vi "hamming encoder.vi"(10 "number of control bits":i32, 11 "message":u8) -> (3 "output array":bool[](array[boolean]))   [LabVIEW 2025]
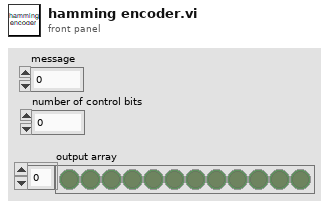
[diagram p1: front panel]
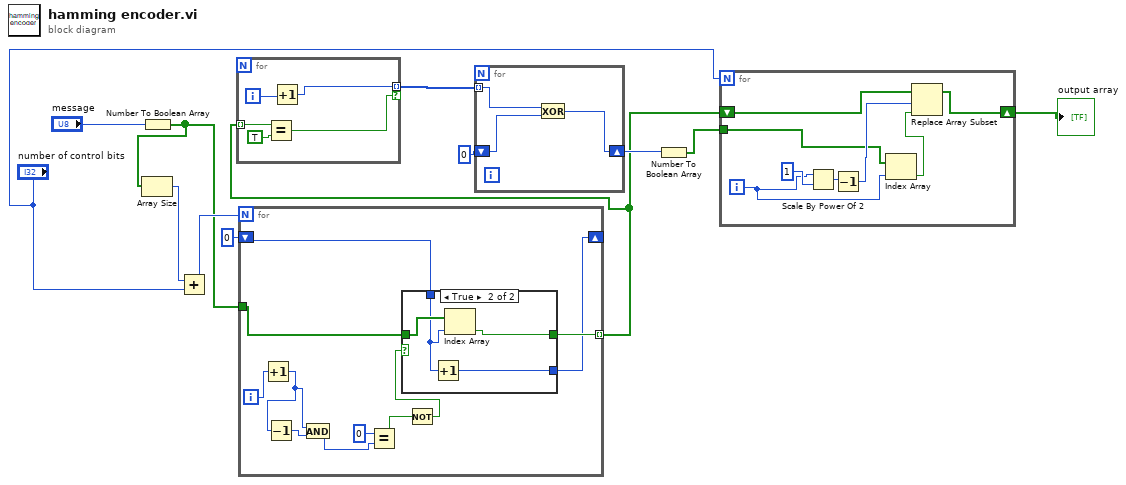
[diagram p0: block diagram]
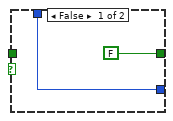
[diagram p2: hidden frame]
diagram:
  n1 = Number To Boolean Array(number="message") -> (Boolean array=w2:bool[])
  n2 = Array Size(array=w2) -> (size(s)=w7:i32)
  n3 = Add(x=w7, y="number of control bits") -> (x+y=w8:i32)
  n4 = for {
    N: w8 -> [_]
    tunnel: w2 -> [w20]
    tunnel: [w21] -> w1 mode=indexing
    shift-right: [w18] -> _
    shift-left: 0 -> [w19]
    i -> [w17]
    n5 = Increment(x=w17) -> (x+1=w13:i32)
    n6 = Decrement(x=w13) -> (x-1=w14:i32)
    n7 = And(x=w13, y=w14) -> (x .and. y?=w23:i32)
    n8 = Equal?(x=0, y=w23) -> (x = y?=w16:bool)
    n9 = Not(x=w16) -> (.not. x?=w15:bool)
    n10 = case shown="True" w15 {
      tunnel: [FALSE w28] -> w21
      tunnel: w20 -> [_ w29]
      tunnel: w19 -> [w24 w27]
      tunnel: [w24 w26] -> w18
      frame False {
      }
      frame True {
        n11 = Increment(x=w27) -> (x+1=w26:i32)
        n12 = Index Array(array=w29, index=w27) -> (element=w28:bool)
      }
    }
  }
  n13 = for {
    tunnel: w1 -> [w33] mode=indexing
    tunnel: [w31] -> w11 mode=indexing if=w30
    i -> [w34]
    n14 = Equal?(x=w33, y=TRUE) -> (x = y?=w30:bool)
    n15 = Increment(x=w34) -> (x+1=w31:i32)
  }
  n16 = for {
    shift-right: [w35] -> w9
    shift-left: 0 -> [w36]
    tunnel: w11 -> [w37] mode=indexing
    n17 = Exclusive Or(1:w36, 2:w37) -> (0:w35:i32)
  }
  n18 = Number To Boolean Array(number=w9) -> (Boolean array=w6:bool[])
  n19 = for {
    N: "number of control bits" -> [_]
    tunnel: w6 -> [w41]
    shift-right: [w44] -> w4
    shift-left: w1 -> [w45]
    i -> [w38]
    n20 = Scale By Power Of 2(n=w38, x=i16 1 ("n")) -> (x*2^n=w43:i16)
    n21 = Decrement(x=w43) -> (x-1=w42:i16)
    n22 = Index Array(array=w41, index=w38) -> (element=w40:bool)
    n23 = Replace Array Subset(array=w45, new element=w40, index=w42) -> (w44:bool[])
  }
  "output array" <- w4
